vi "test tools list array shapes.vi"(8 "error in (no error)":errorcluster) -> (0 "error out":errorcluster, 2 "tool entry":string, 3 "body":string)   [LabVIEW 2020, in "MCP Server tests.lvlib"]
doc: "tools/list must describe array inputs with items and the type of their elements, also for shapes beyond 1D arrays of plain numbers, strings and Booleans. fake_tool_array_shapes is found in the tools/list answer by its MCP name, and each of these array inputs gets its own assertion: array3d, a 3D array of DBL, must be described as an array of arrays of arrays of numbers - items.type and items.items.type are array and items.items.items.type is number. patharray, a 1D array of paths, enumarray, a 1D array of a U16 enum, and clusterarray, a 1D array of clusters, must each have items with a non-empty type. The request is sent with the LabVIEW HTTP Client directly."
uses:
  MCP Server tests.lvlib
  06ffe2ea-474a-416a-9b98-ff53180db269.vi
  <vilib>/JDP Science/JSONtext/Next JSON Value.vi
  <vilib>/JDP Science/JSONtext/String Subset.vi
  <vilib>/JDP Science/JSONtext/Parsing/Advance past next JSON Value (inlined COPY).vi
  <vilib>/JDP Science/JSONtext/Parsing/Advance past whitespace.vi
  <vilib>/JDP Science/JSONtext/Parsing/Advance past String.vi
  <vilib>/JDP Science/JSONtext/Parsing/Advance past Number.vi
  <vilib>/JDP Science/JSONtext/Parsing/Advance past Line Ending.vi
  <vilib>/JDP Science/JSONtext/Parsing/Parse Full Path or Item Name.vi
  <vilib>/JDP Science/JSONtext/Parsing/Advance past Array.vi
  <vilib>/JDP Science/JSONtext/Parsing/Advance past Object.vi
  <vilib>/JDP Science/JSONtext/support/Error Cluster From Code.vi
  <vilib>/JDP Science/JSONtext/Offset/Find Item Locations by Path.vi
  <vilib>/JDP Science/JSONtext/JSON text to Variant.vi
  <vilib>/JDP Science/JSONtext/LVClass Serializer/JSONtext LVClass Serializer.lvclass
  <vilib>/addons/_JKI Toolkits/Caraya/classes/Test/Test.lvclass
  <vilib>/JDP Science/JSONtext/JSONtext.lvlib
  <vilib>/addons/_JKI Toolkits/Caraya/classes/Assert/Assert.lvclass
panel:
  out "lookup error":errorcluster
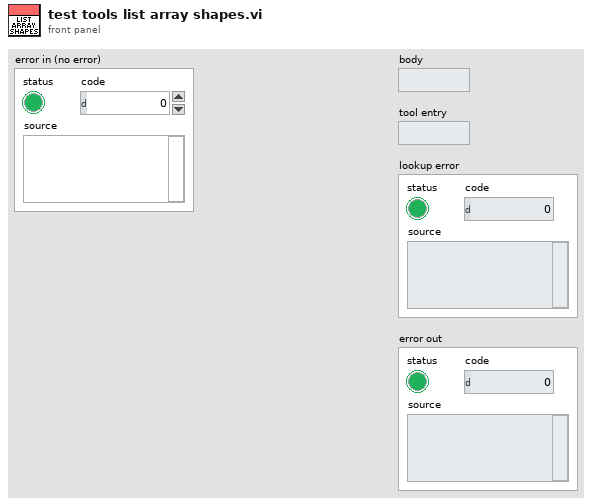
[diagram p1: front panel]
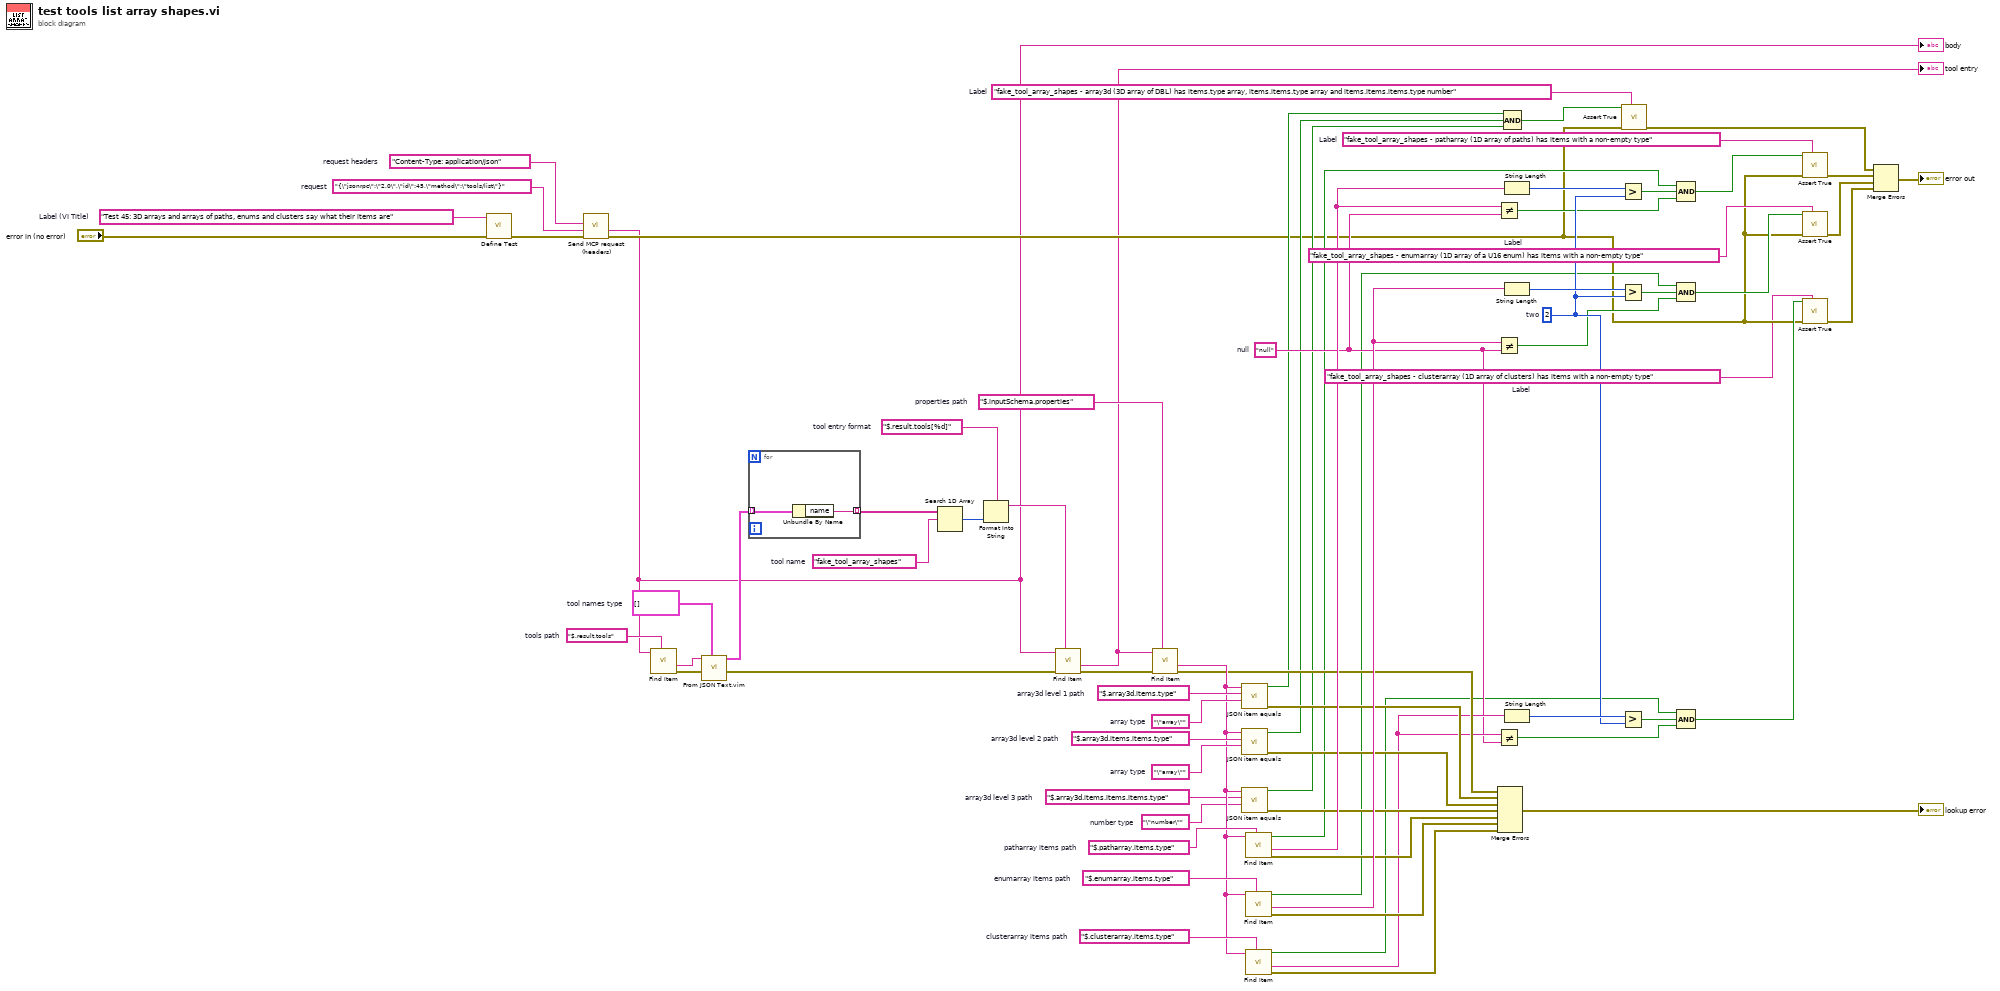
[diagram p0: block diagram]
diagram:
  w50 = "\"array\""  # array type
  w70 = "Content-Type: application/json"  # request headers
  w9 = "fake_tool_array_shapes - clusterarray (1D array of clusters) has items with a non-empty type"  # Label
  w52 = "$.clusterarray.items.type"  # clusterarray items path
  w12 = "fake_tool_array_shapes - enumarray (1D array of a U16 enum) has items with a non-empty type"  # Label
  w53 = "$.enumarray.items.type"  # enumarray items path
  w14 = "fake_tool_array_shapes - patharray (1D array of paths) has items with a non-empty type"  # Label
  w54 = "$.patharray.items.type"  # patharray items path
  w25 = "fake_tool_array_shapes - array3d (3D array of DBL) has items.type array, items.items.type array and items.items.items.type number"  # Label
  w45 = "\"number\""  # number type
  w48 = "\"array\""  # array type
  w46 = "$.array3d.items.items.items.type"  # array3d level 3 path
  w49 = "$.array3d.items.items.type"  # array3d level 2 path
  w51 = "$.array3d.items.type"  # array3d level 1 path
  w27 = 2  # two
  w34 = "null"  # null
  w55 = "$.inputSchema.properties"  # properties path
  w59 = "$.result.tools[%d]"  # tool entry format
  w61 = "fake_tool_array_shapes"  # tool name
  w64 = cluster{"name":string}[] []  # tool names type
  w67 = "$.result.tools"  # tools path
  w69 = "{\"jsonrpc\":\"2.0\",\"id\":45,\"method\":\"tools/list\"}"  # request
  w72 = "Test 45: 3D arrays and arrays of paths, enums and clusters say what their items are"  # Label (VI Title)
  n1 = call <vilib>:"Define Test.vi"("error in (no error)"="error in (no error)", "Label (VI Title)"=w72) -> ("error out"=w68:errorcluster)  [unwired: 8 in, 1 out]
  n2 = call "Send MCP request (headers).vi"("error in (no error)"=w68, "request"=w69, "request headers"=w70) -> ("error out"=w10:errorcluster, "response"=w4:string)  [unwired: 5 in, 2 out]
  "body" <- w4
  n3 = call <vilib>:"Find Item.vi"("$Path or Item Name"=w67, "JSON"=w4) -> ("error out"=w65:errorcluster, "<JSON>"=w66:string)  [unwired: 6 in, 2 out]
  n4 = call "From JSON Text.vim"("Data Type and Default Value"=w64, "error in (no error)"=w65, "JSON"=w66) -> ("error out"=w58:errorcluster, "Data out"=w63:cluster{"name":string}[])  [unwired: 7 in]
  n5 = for {
    tunnel: w63 -> [w74] mode=indexing
    tunnel: [w73] -> w62 mode=indexing
    n6 = Unbundle By Name(w74) -> ("name"=w73:string)
  }
  n7 = Search 1D Array(1D array=w62, element=w61) -> (index of element=w60:i32)  [unwired: 1 in]
  n8 = Format Into String(format string=w59, w60) -> (resulting string=w57:string)  [unwired: 2 in, 1 out]
  n9 = call <vilib>:"Find Item.vi"("$Path or Item Name"=w57, "error in (no error)"=w58, "JSON"=w4) -> ("error out"=w56:errorcluster, "<JSON>"=w3:string)  [unwired: 5 in, 2 out]
  "tool entry" <- w3
  n10 = call <vilib>:"Find Item.vi"("$Path or Item Name"=w55, "error in (no error)"=w56, "JSON"=w3) -> ("error out"=w42:errorcluster, "<JSON>"=w47:string)  [unwired: 5 in, 2 out]
  n11 = call "JSON item equals.vi"("expected"=w50, "path"=w51, "JSON"=w47) -> ("error out"=w41:errorcluster, "equal?"=w33:bool)  [unwired: 6 in, 1 out]
  n12 = call "JSON item equals.vi"("expected"=w48, "path"=w49, "JSON"=w47) -> ("error out"=w40:errorcluster, "equal?"=w32:bool)  [unwired: 6 in, 1 out]
  n13 = call "JSON item equals.vi"("expected"=w45, "path"=w46, "JSON"=w47) -> ("error out"=w39:errorcluster, "equal?"=w31:bool)  [unwired: 6 in, 1 out]
  n14 = call <vilib>:"Find Item.vi"("$Path or Item Name"=w54, "JSON"=w47) -> ("error out"=w38:errorcluster, "<JSON>"=w44:string, "Found"=w24:bool)  [unwired: 6 in, 1 out]
  n15 = call <vilib>:"Find Item.vi"("$Path or Item Name"=w53, "JSON"=w47) -> ("error out"=w37:errorcluster, "<JSON>"=w43:string, "Found"=w21:bool)  [unwired: 6 in, 1 out]
  n16 = call <vilib>:"Find Item.vi"("$Path or Item Name"=w52, "JSON"=w47) -> ("error out"=w36:errorcluster, "<JSON>"=w35:string, "Found"=w18:bool)  [unwired: 6 in, 1 out]
  n17 = Not Equal?(x=w44, y=w34) -> (x != y?=w22:bool)
  n18 = Not Equal?(x=w43, y=w34) -> (x != y?=w19:bool)
  n19 = Not Equal?(x=w35, y=w34) -> (x != y?=w16:bool)
  n20 = Merge Errors(w42, w41, w40, w39, w38, w37, w36) -> (→"lookup error":errorcluster)
  n21 = Compound Arithmetic op=AND(w33, w32, w31) -> (w26:bool)
  n22 = String Length(string=w44) -> (length=w30:i32)
  n23 = String Length(string=w43) -> (length=w29:i32)
  n24 = String Length(string=w35) -> (length=w28:i32)
  n25 = Greater?(x=w30, y=w27) -> (0:w23:bool)
  n26 = Greater?(x=w29, y=w27) -> (0:w20:bool)
  n27 = Greater?(x=w28, y=w27) -> (0:w17:bool)
  n28 = call <vilib>:"Assert True.vi"("Label"=w25, "error in (no error)"=w10, "True?"=w26) -> ("error out"=w8:errorcluster)  [unwired: 7 in, 1 out]
  n29 = Compound Arithmetic op=AND(w24, w23, w22) -> (w15:bool)
  n30 = Compound Arithmetic op=AND(w21, w20, w19) -> (w13:bool)
  n31 = Compound Arithmetic op=AND(w18, w17, w16) -> (w11:bool)
  n32 = call <vilib>:"Assert True.vi"("Label"=w14, "error in (no error)"=w10, "True?"=w15) -> ("error out"=w7:errorcluster)  [unwired: 7 in, 1 out]
  n33 = call <vilib>:"Assert True.vi"("Label"=w12, "error in (no error)"=w10, "True?"=w13) -> ("error out"=w6:errorcluster)  [unwired: 7 in, 1 out]
  n34 = call <vilib>:"Assert True.vi"("Label"=w9, "error in (no error)"=w10, "True?"=w11) -> ("error out"=w5:errorcluster)  [unwired: 7 in, 1 out]
  n35 = Merge Errors(w8, w7, w6, w5) -> (→"error out":errorcluster)
